vi "Construct.vi"(4 "Stale (F)":bool, 6 "Properties":variant, 8 "error in (no error)":errorcluster, 9 "Initial Value":variant, 10 "Name":string, 11 "Tag in":refnum<class "Tag.lvclass">) -> (0 "error out":errorcluster, 3 "Tag out":refnum<class "Tag.lvclass">)   [LabVIEW 2020, in "Tag Engine Core.lvlib" / "Tag.lvclass"]
doc: "_SubVI_\nInitializes the Tag object.\nThe input initial value will define the type.\n\nThe input Tag name is sanitized. Illegal characters are replaced with underscores.\n\nAdditional properties can be passed in as attributes of the properties varriant."
uses:
  Tag.lvclass
  Types/SetRequest Cluster.ctl
  <vilib>/Utility/Data Type/Type Definitions/Data Type.ctl
  Types/ValChange Cluster.ctl
  Tag.lvclass/Tag.ctl
  <vilib>/Utility/error.llb/Error Cluster From Error Code.vi
  <vilib>/ErrorRing/Error Ring.xnode
  Tag Engine Core.lvlib
  <vilib>/Utility/Data Type/NI_Data Type.lvlib
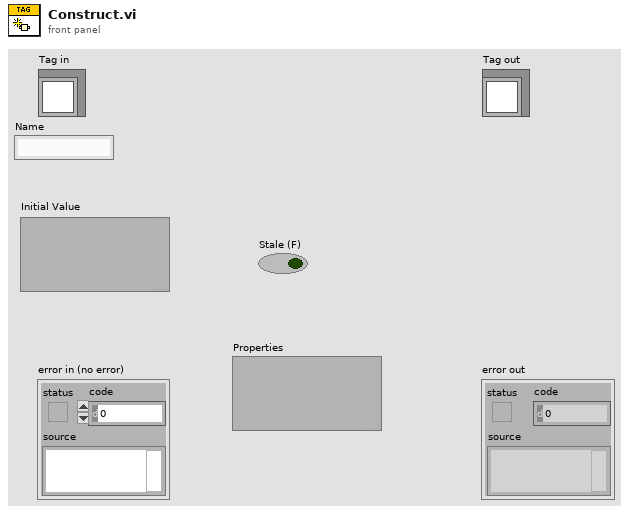
[diagram p1: front panel]
types:
  T1 = typedef "Tag Engine Core.lvlib/SetRequest Cluster.ctl" = cluster{"Tag Name":string, "Type":T2, "Old Value":variant, "Old Time Stamp":timestamp, "Req Value":variant, "Req Time Stamp":timestamp, "Callback":refnum<notifier>, "Synchronous (F)":bool}
  T2 = typedef "NI_Data Type.lvlib/Data Type.ctl" = enum8{"Invalid Type", "Void", "I8", "I16", "I32", "I64", "U8", "U16", "U32", "U64", "Single Float", "Double Float", "Extended Float", "Single Complex", "Double Complex", "Extended Complex", "Enum U8", "Enum U16", "Enum U32", "Enum U64", "Single Float With Unit", "Double Float With Unit", "Extended Float With Unit", "Single Complex with Unit", "Double Complex with Unit", "Extended Complex with Unit", "Boolean", "String", "Path", "Picture", "Tag", "Array", "Cluster", "Variant", "LV Variant", "Waveform", "Timestamp", "Digital Waveform", "Digital Data", "ExpressData", "Refnum", "External Data", "VI", "Poly VI", "LabVIEW Class Instance", "Fixed Point", "Set Collection", "Map Collection"}
  T3 = typedef "Tag Engine Core.lvlib/ValChange Cluster.ctl" = cluster{"Tag Name":string, "Type":T2, "Old Value":variant, "Old Time Stamp":timestamp, "New Value":variant, "New Time Stamp":timestamp}
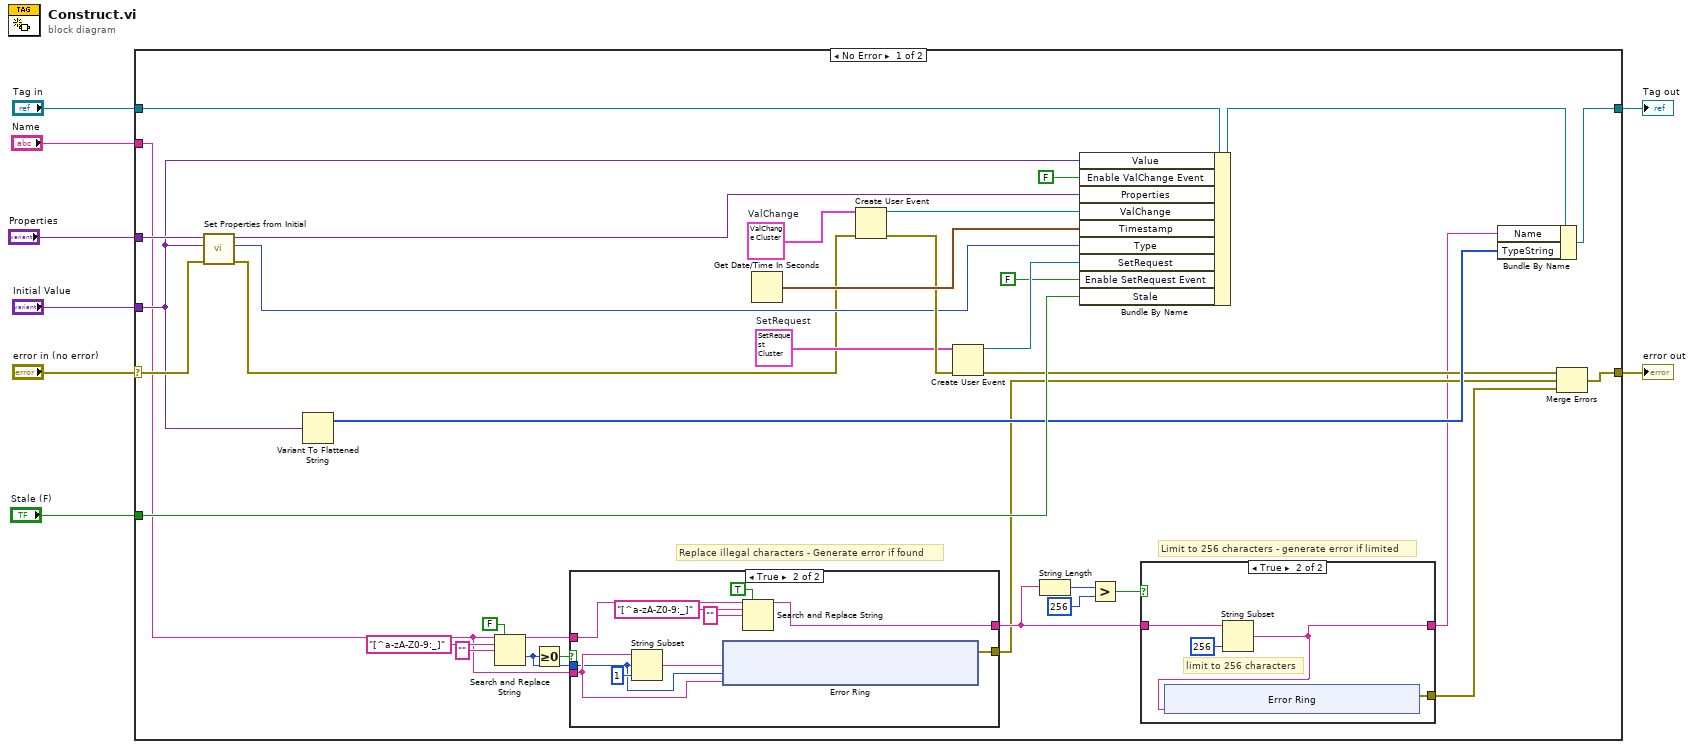
[diagram p0: block diagram]
diagram:
  n1 = case shown="No Error" "error in (no error)" {
    selector: "error in (no error)" -> [w31 w77]
    tunnel: [w10 w77] -> w7
    tunnel: [w28 w76] -> w5
    tunnel: "Tag in" -> [w42 w76]
    tunnel: "Name" -> [w19 _]
    tunnel: "Initial Value" -> [w26 _]
    tunnel: "Properties" -> [w34 _]
    tunnel: "Stale (F)" -> [w30 _]
    frame No Error {
      w37 = T1 {"Tag Name"="", "Type"=enum."Variant", "Old Value"=variant, "Old Time Stamp"=timestamp(0 s since 1904-01-01), "Req Value"=variant, "Req Time Stamp"=timestamp(0 s since 1904-01-01), "Callback"=refnum, "Synchronous (F)"=FALSE}  # SetRequest
      w43 = T3 {"Tag Name"="", "Type"=enum."Variant", "Old Value"=variant, "Old Time Stamp"=timestamp(0 s since 1904-01-01), "New Value"=variant, "New Time Stamp"=timestamp(0 s since 1904-01-01)}  # ValChange
      # "Limit to 256 characters - generate error if limited"
      # "Replace illegal characters - Generate error if found"
      n2 = call "Set Properties from Initial.vi"("error in(no error)"=w31, "Initial Value"=w26, "Properties in"=w34) -> ("error out"=w14:errorcluster, "type"=w32:T2, "Properties out"=w33:variant)  [unwired: 6 in]
      n3 = Variant To Flattened String(Variant=w26) -> (1:w27:i16[])  [unwired: 1 out]
      n4 = Search and Replace String(replace all?=FALSE ("replace all? (F)"), input string=w19, search string="[^a-zA-Z0-9:_]", replace string="" ("replace string (\"\")")) -> (result string=w21:string, offset past replacement=w22:i32)  [unwired: 4 in, 2 out]
      n5 = Greater Or Equal To 0?(x=w22) -> (x >= 0?=w23:bool)
      n6 = case shown="True" w23 {
        tunnel: w19 -> [w56 w64]
        tunnel: w22 -> [_ w62]
        tunnel: w21 -> [_ w58]
        tunnel: [_ w63] -> w13
        tunnel: [w56 w57] -> w15
        frame False {
        }
        frame True {
          n7 = String Subset(string=w64, offset (0)=w62, length (rest)=1 ("length (rest)")) -> (substring=w65:string)
          n8 = xnode "Error Ring"("parameter 0"=w65, "parameter 1"=w62, "parameter 2"=w64) -> ("error out"=w63:errorcluster)
          n9 = Search and Replace String(replace all?=TRUE ("replace all? (F)"), input string=w58, search string="[^a-zA-Z0-9:_]", replace string="" ("replace string (\"\")")) -> (result string=w57:string)  [unwired: 4 in, 3 out]
        }
      }
      n10 = Get Date/Time In Seconds() -> (seconds since 1Jan1904=w39:timestamp)
      n11 = Create User Event(user event datatype=w43, error in=w14) -> (user event=w41:refnum<user-event>, error out=w38:errorcluster)
      n12 = Create User Event(user event datatype=w37, error in=w38) -> (user event=w36:refnum<user-event>, error out=w11:errorcluster)
      n13 = String Length(string=w15) -> (length=w18:i32)
      n14 = Bundle By Name(cluster=w42, "Value"=w26, "Enable ValChange Event"=FALSE, "Properties"=w33, "ValChange"=w41, "Timestamp"=w39, "Type"=w32, "SetRequest"=w36, "Enable SetRequest Event"=FALSE, "Stale"=w30) -> (w29:refnum<class "Tag.lvclass">)
      n15 = Greater?(x=w18, y=256) -> (0:w16:bool)
      n16 = case shown="True" w16 {
        tunnel: w15 -> [w44 w47]
        tunnel: [w44 w46] -> w9
        tunnel: [_ w45] -> w12
        frame False {
        }
        frame True {
          # "limit to 256 characters"
          n17 = String Subset(string=w47, length (rest)=256 ("length (rest)")) -> (substring=w46:string)  [unwired: 1 in]
          n18 = xnode "Error Ring"("parameter 0"=w46) -> ("error out"=w45:errorcluster)
        }
      }
      n19 = Bundle By Name(cluster=w29, "Name"=w9, "TypeString"=w27) -> (w28:refnum<class "Tag.lvclass">)
      n20 = Merge Errors(w11, w13, w12) -> (w10:errorcluster)
    }
    frame Error {
    }
  }
  "error out" <- w7
  "Tag out" <- w5
